vi "select 8000A LTE Target.vi"(8 "error in (no error)":errorcluster, 11 "LTE in":refnum<class "LTE.lvclass">) -> (0 "error out":errorcluster, 3 "LTE out":refnum<class "LTE.lvclass">)   [LabVIEW 2023, in "ANRITSU Call Box.lvlib" / "LTE.lvclass"]
uses:
  LTE.lvclass
  Type Definition/Call Device - Protocol Type Selector.ctl
  LTE.lvclass/LTE.ctl
  ANRITSU Call Box.lvlib
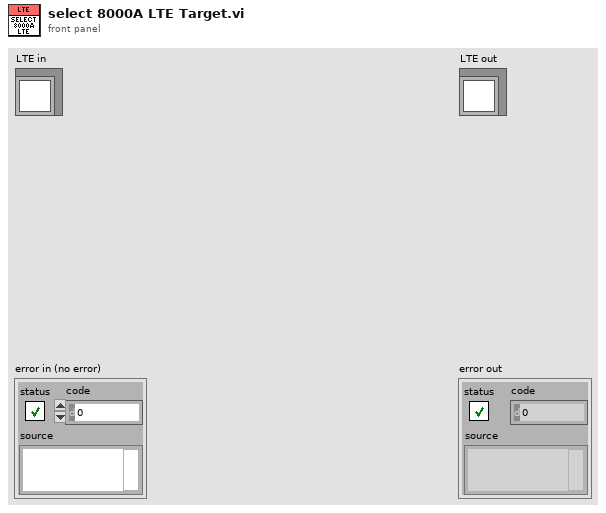
[diagram p1: front panel]
types:
  T1 = typedef "ANRITSU Call Box.lvlib/Call Device - Protocol Type Selector.ctl" = enum16{"8000A - NR", "8000A - LTE", "882xC - LTE"}
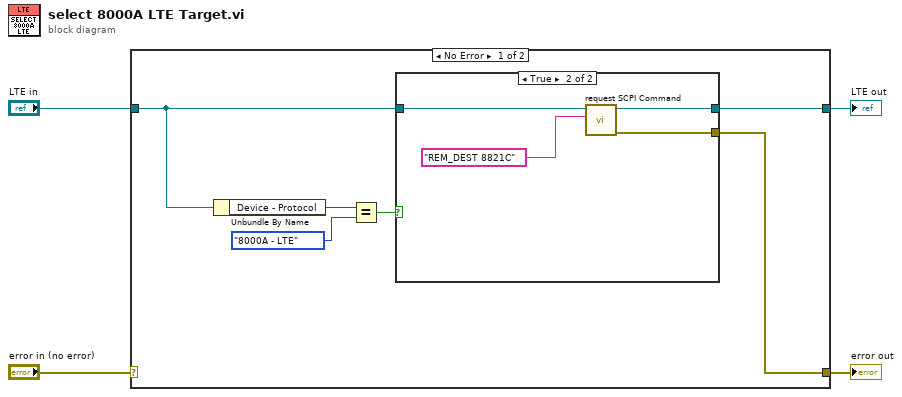
[diagram p0: block diagram]
diagram:
  n1 = case shown="No Error" "error in (no error)" {
    selector: "error in (no error)" -> [_ w17]
    tunnel: [w9 w17] -> w3
    tunnel: [w10 w16] -> w1
    tunnel: "LTE in" -> [w8 w16]
    frame No Error {
      n2 = Unbundle By Name(w8) -> ("Device - Protocol"=w7:T1)
      n3 = Equal?(x=w7, y=Call_Device_-_Protocol_Type_Selector."8000A - LTE") -> (x = y?=w5:bool)
      n4 = case shown="True" w5 {
        tunnel: [w11 w14] -> w10
        tunnel: [_ w13] -> w9
        tunnel: w8 -> [w11 w12]
        frame False {
        }
        frame True {
          n5 = call "request SCPI Command.vi"("SCPI Command"="REM_DEST 8821C" ("write buffer"), "LTE in"=w12) -> ("error out"=w13:errorcluster, "LTE out"=w14:refnum<class "LTE.lvclass">)  [unwired: 8 in]
        }
      }
    }
    frame Error {
    }
  }
  "error out" <- w3
  "LTE out" <- w1
